vi "Initialization.vi"(8 "error in":errorcluster, 9 "UI Refs":T1, 10 "user event":T2, 11 "Frequency Response":refnum<class "H1 Frequency Response.lvclass">) -> (0 "error out":errorcluster, 3 "Frequency Response":refnum<class "H1 Frequency Response.lvclass">)   [LabVIEW 2025, in "H1 Plotter.lvlib" / "H1 Frequency Response.lvclass"]
uses:
  H1 Frequency Response.lvclass
  Users/Public/Documents/Sandia National Labs/TSS Plugin/CEF.lvlibp/Node/UserEventRef.ctl
  <vilib>/Utility/miscctls.llb/LVAnnotationListTypeDef.ctl
  H1 Frequency Response.lvclass/H1 Frequency Response.ctl
  Users/Public/Documents/Sandia National Labs/TSS Plugin/Tests/XY Plotter.lvlibp/XY  Plotter/XY Plotter.lvclass
  Users/Public/Documents/Sandia National Labs/TSS Plugin/CEF.lvlibp/Node/CEF_Node.lvclass
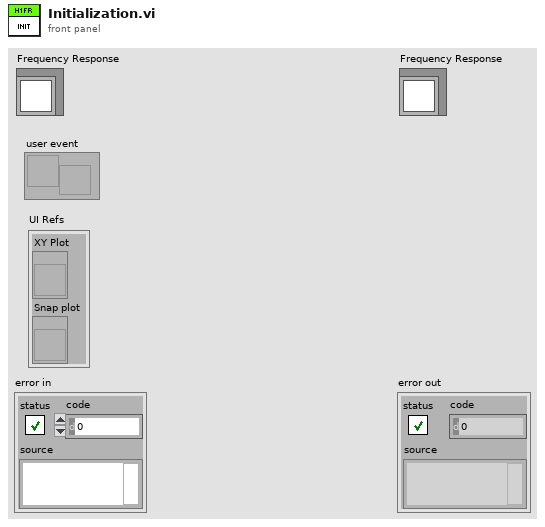
[diagram p1: front panel]
types:
  T1 = cluster{"XY Plot":refnum<vi>, "Snap plot":refnum<vi>}
  T2 = typedef "CEF.lvlibp/CEF_Node.lvclass/UserEventRef.ctl" = refnum<user-event>
  T3 = typedef "LVAnnotationListTypeDef.ctl" = cluster{"Name":string, "Color":u32, "Style":u8, "Point Style":u8, "Name Visible":bool, "Allow Drag":bool, "Annotation Mode":u32, "Plot":i32, "Index":i32, "Position":cluster{"X":dbl, "Y":dbl}, "X Scale":u32, "Y Scale":u32, "Show Arrow":bool, "Lock Name":bool, "Plot Area":i32, "Label Offset":cluster{"X":dbl, "Y":dbl}}[]
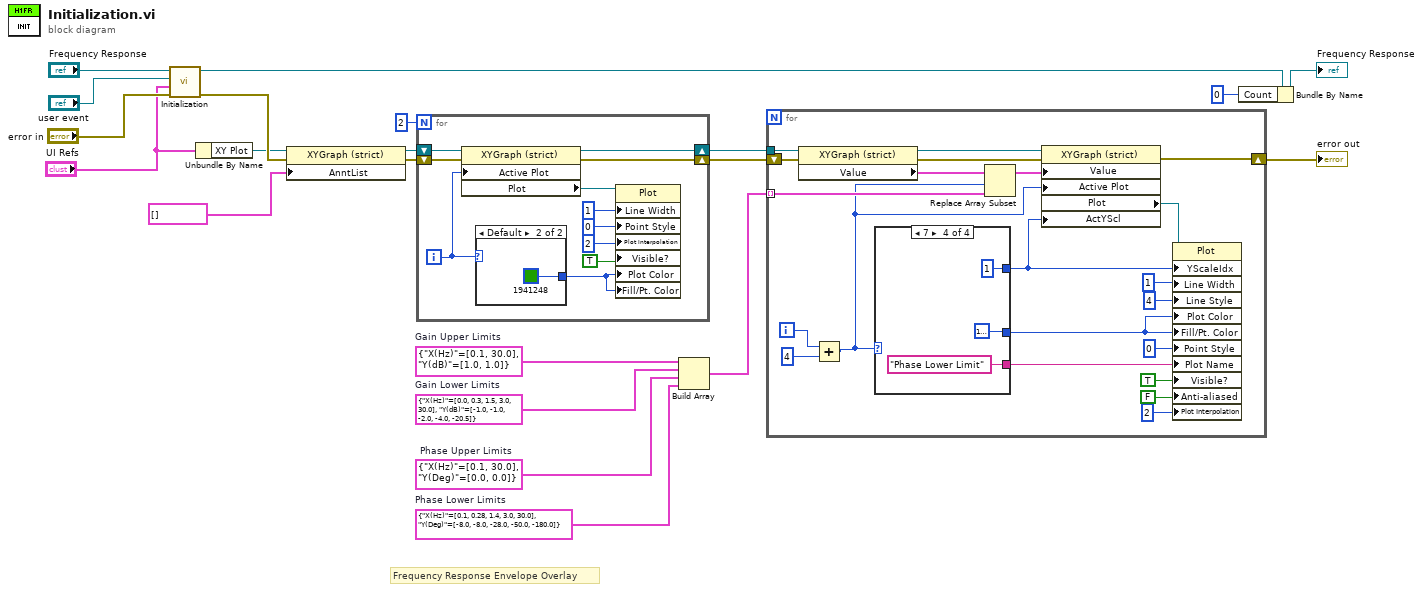
[diagram p0: block diagram]
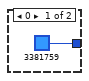
[diagram p2: hidden frame]
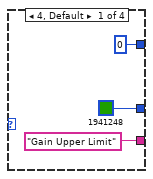
[diagram p3: hidden frame]
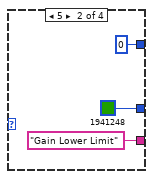
[diagram p4: hidden frame]
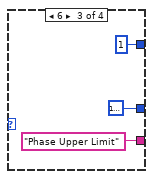
[diagram p5: hidden frame]
diagram:
  w17 = cluster{"X(Hz)":dbl[], "Y(Deg)":dbl[]} {"X(Hz)"=[0.1, 0.28, 1.4, 3.0, 30.0], "Y(Deg)"=[-8.0, -8.0, -28.0, -50.0, -180.0]}  # Phase Lower Limits
  w16 = cluster{"X(Hz)":dbl[], "Y(Deg)":dbl[]} {"X(Hz)"=[0.1, 30.0], "Y(Deg)"=[0.0, 0.0]}  # Phase Upper Limits
  w15 = cluster{"X(Hz)":dbl[], "Y(dB)":dbl[]} {"X(Hz)"=[0.0, 0.3, 1.5, 3.0, 30.0], "Y(dB)"=[-1.0, -1.0, -2.0, -4.0, -20.5]}  # Gain Lower Limits
  w14 = cluster{"X(Hz)":dbl[], "Y(dB)":dbl[]} {"X(Hz)"=[0.1, 30.0], "Y(dB)"=[1.0, 1.0]}  # Gain Upper Limits
  # "Frequency Response Envelope Overlay"
  n1 = call-parent "Initialization.vi"("error in"="error in", "UI Refs"="UI Refs", "user event"="user event", "XY Plotter"="Frequency Response") -> ("error out"=w8:errorcluster, "XY Plotter out"=w12:refnum<class "H1 Frequency Response.lvclass">)  [unwired: 6 in]
  n2 = Unbundle By Name("UI Refs") -> ("XY Plot"=w3:refnum<vi>)
  n3 = property class="XYGraph (strict)"(reference=w3, error in=w8, "AnntList"=T3 [] ("Annotation List")) -> (reference out=w2:refnum<vi>, error out=w4:errorcluster)
  n4 = for {
    N: 2 -> [_]
    shift-right: [w23] -> w7
    shift-left: w4 -> [w27]
    shift-right: [w22] -> w9
    shift-left: w2 -> [w32]
    i -> [w25]
    n5 = property class="XYGraph (strict)"(reference=w32, error in=w27, "Active Plot"=w25) -> (reference out=w22:refnum<vi>, error out=w23:errorcluster, "Plot"=w28:refnum<vi>)
    n6 = case shown="Default" w25 {
      tunnel: [u32 3381759 ("Plot Color") u32 1941248 ("Plot Color")] -> w24
      frame 0 {
      }
      frame Default {
      }
    }
    n7 = property class="Plot"(reference=w28, "Line Width"=u8 1, "Point Style"=u8 0, "Plot Interpolation"=u8 2, "Visible?"=TRUE ("Visible"), "Plot Color"=w24, "Fill/Pt. Color"=w24) -> ()  [unwired: 1 in, 2 out]
  }
  n8 = Build Array(w14, w15, w16, w17) -> (w13:cluster{"X(Hz)":dbl[], "Y(Deg)":dbl[]}[])
  n9 = for {
    tunnel: w13 -> [w55] mode=indexing
    tunnel: w9 -> [w39]
    shift-right: [w35] -> w6
    shift-left: w7 -> [w36]
    i -> [w44]
    n10 = property class="XYGraph (strict)"(reference=w39, error in=w36) -> (reference out=w38:refnum<vi>, error out=w40:errorcluster, "Value"=w37:cluster{"Wavenumber":dbl[], "Data":dbl[]}[])
    n11 = Add(x=w44, y=4) -> (x+y=w42:i32)
    n12 = case shown="7" w42 {
      tunnel: [u32 1941248 ("Plot.Plot Color") u32 1941248 ("Plot.Plot Color") u32 16777224 ("Plot.Plot Color") u32 16777224 ("Plot.Plot Color")] -> w54
      tunnel: ["Gain Upper Limit" ("Plot Name") "Gain Lower Limit" ("Plot Name") "Phase Upper Limit" ("Plot Name") "Phase Lower Limit" ("Plot Name")] -> w50
      tunnel: [u8 0 ("Line Width") u8 0 ("Line Width") u8 1 ("Line Width") u8 1 ("Line Width")] -> w41
      frame 4, Default {
      }
      frame 5 {
      }
      frame 6 {
      }
      frame 7 {
      }
    }
    n13 = Replace Array Subset(array=w37, new element=w55, index=w42) -> (w52:cluster{"Wavenumber":dbl[], "Data":dbl[]}[])
    n14 = property class="XYGraph (strict)"(reference=w38, error in=w40, "Value"=w52, "Active Plot"=w42, "ActYScl"=w41) -> (error out=w35:errorcluster, "Plot"=w53:refnum<vi>)  [unwired: 1 out]
    n15 = property class="Plot"(reference=w53, "YScaleIdx"=w41, "Line Width"=u8 1, "Line Style"=u8 4, "Plot Color"=w54, "Fill/Pt. Color"=w54, "Point Style"=u8 0, "Plot Name"=w50, "Visible?"=TRUE ("Visible"), "Anti-aliased"=FALSE, "Plot Interpolation"=u8 2) -> ()  [unwired: 1 in, 2 out]
  }
  "error out" <- w6
  n16 = Bundle By Name(cluster=w12, "Count"=0) -> (→"Frequency Response":refnum<class "H1 Frequency Response.lvclass">)
